vi "Add String for Path Control.vi"(0 "String Controls in":refnum<vi>, 1 "String Names in":string[](array[string]), 2 "Controls Ref IN":refnum<vi>[](array[refnum]), 5 "Path Refnum":refnum<vi>, 7 "vi reference":refnum<vi>, 11 "error in (no error)":errorcluster) -> (4 "Controls Ref Out":refnum<vi>[](array[refnum]), 6 "String Names Out":string[](array[string]), 15 "error out":errorcluster)   [LabVIEW 2021, in "Migrator.lvlib"]
uses:
  Migrator.lvlib
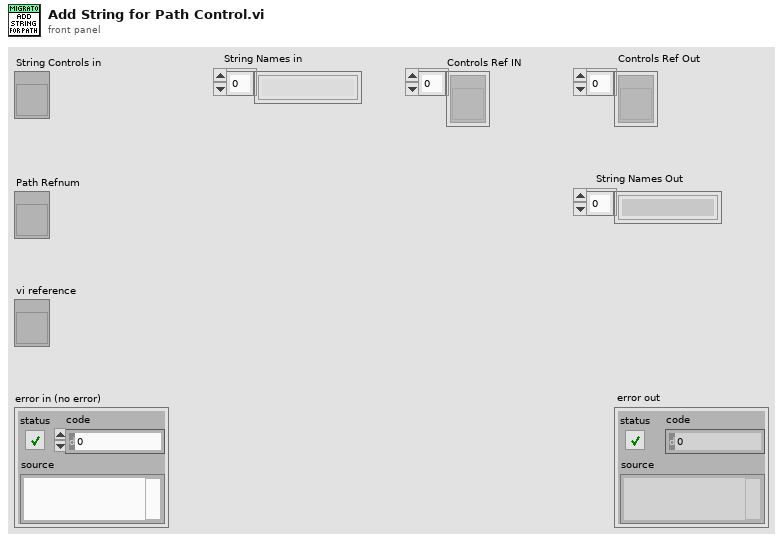
[diagram p1: front panel]
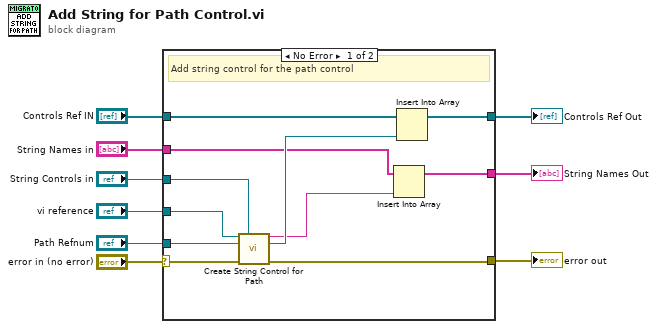
[diagram p0: block diagram]
diagram:
  n1 = case shown="No Error" "error in (no error)" {
    selector: "error in (no error)" -> [w20 w23]
    tunnel: "vi reference" -> [w19 _]
    tunnel: "Path Refnum" -> [w18 _]
    tunnel: "String Controls in" -> [w17 _]
    tunnel: "Controls Ref IN" -> [w16 w22]
    tunnel: [w14 w22] -> w4
    tunnel: [w13 w23] -> w3
    tunnel: "String Names in" -> [w11 w21]
    tunnel: [w10 w21] -> w1
    frame No Error {
      # "Add string control for the path control"
      n2 = call "Create String Control for Path.vi"("VI Refnum"=w19, "Typedef Cluster"=w17, "Path Refnum"=w18, "error in (no error)"=w20) -> ("Reference String"=w12:string, "String ctl ref"=w15:refnum<vi>, "error out"=w13:errorcluster)  [unwired: 9 in]
      n3 = Insert Into Array(array=w11, new element=w12) -> (w10:string[])  [unwired: 1 in]
      n4 = Insert Into Array(array=w16, new element=w15) -> (w14:refnum<vi>[])  [unwired: 1 in]
    }
    frame Error {
    }
  }
  "Controls Ref Out" <- w4
  "error out" <- w3
  "String Names Out" <- w1
